vi "Set Annotation.vi"(8 "error in":errorcluster, 9 "XY Position":T1 caption="Position", 10 "Active Plot":u32, 11 "XY Plot":refnum<vi>) -> (0 "error out":errorcluster, 3 "XY Plot out":refnum<vi>)   [LabVIEW 2025, in "XY Plotter.lvlib" / "XY Plotter.lvclass"]
uses:
  XY Plotter.lvclass
  <vilib>/Utility/miscctls.llb/LVPointDoubleTypeDef.ctl
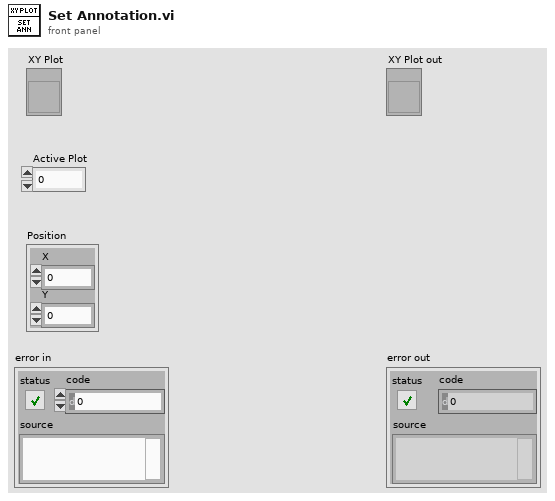
[diagram p1: front panel]
types:
  T1 = typedef "LVPointDoubleTypeDef.ctl" = cluster{"X":dbl, "Y":dbl}
  T2 = cluster{"Name":string, "Color":u32, "Style":u8, "Point Style":u8, "Name Visible":bool, "Allow Drag":bool, "Annotation Mode":u32, "Plot":i32, "Index":i32, "Position":cluster{"X":dbl, "Y":dbl}, "X Scale":u32, "Y Scale":u32, "Show Arrow":bool, "Lock Name":bool, "Plot Area":i32, "Label Offset":cluster{"X":dbl, "Y":dbl}}
  T3 = typedef "LVAnnotationListTypeDef.ctl" = cluster{"Name":string, "Color":u32, "Style":u8, "Point Style":u8, "Name Visible":bool, "Allow Drag":bool, "Annotation Mode":u32, "Plot":i32, "Index":i32, "Position":cluster{"X":dbl, "Y":dbl}, "X Scale":u32, "Y Scale":u32, "Show Arrow":bool, "Lock Name":bool, "Plot Area":i32, "Label Offset":cluster{"X":dbl, "Y":dbl}}[]
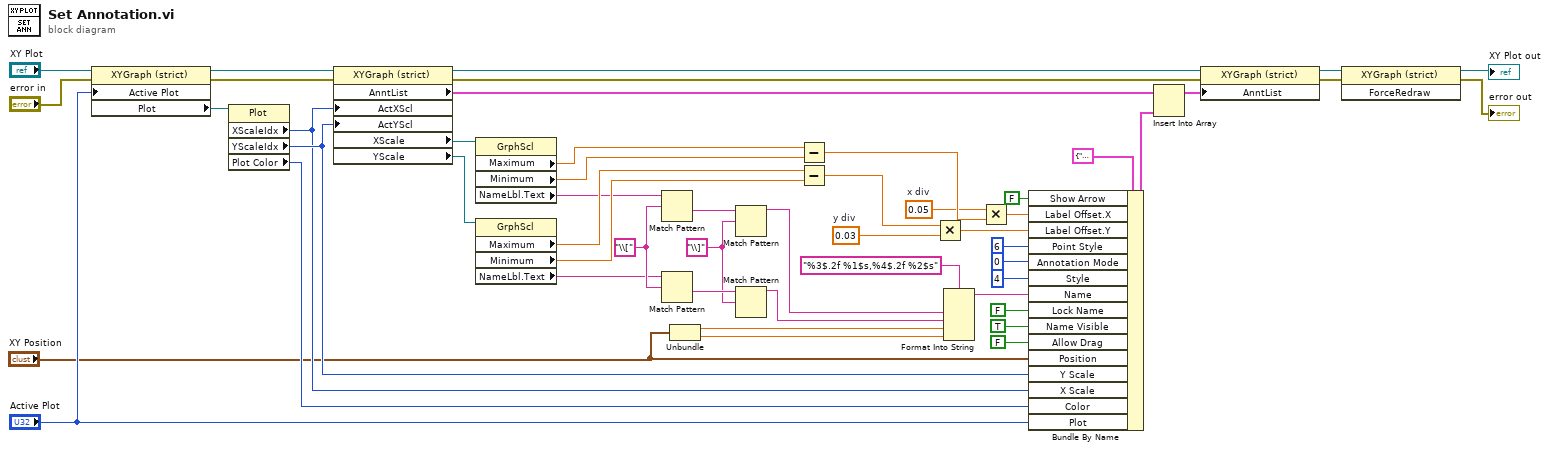
[diagram p0: block diagram]
diagram:
  w11 = "\\]" ("regular expression")
  w8 = "\\[" ("regular expression")
  w9 = 0.03  # y div
  w13 = 0.05  # x div
  n1 = property class="XYGraph (strict)"(reference="XY Plot", error in="error in", "Active Plot"="Active Plot") -> (reference out=w45:refnum<vi>, error out=w43:errorcluster, "Plot"=w35:refnum<vi>)
  n2 = property class="Plot"(reference=w35) -> ("XScaleIdx"=w32:u32, "YScaleIdx"=w33:u32, "Plot Color"=w34:u32)  [unwired: 1 in, 2 out]
  n3 = property class="XYGraph (strict)"(reference=w45, error in=w43, "ActXScl"=w32, "ActYScl"=w33) -> (reference out=w44:refnum<vi>, error out=w42:errorcluster, "AnntList"=w46:T3, "XScale"=w31:refnum<vi>, "YScale"=w30:refnum<vi>)
  n4 = property class="GrphScl"(reference=w31) -> ("Maximum"=w20:dbl, "Minimum"=w21:dbl, "NameLbl.Text"=w7:string)  [unwired: 1 in, 2 out]
  n5 = property class="GrphScl"(reference=w30) -> ("Maximum"=w22:dbl, "Minimum"=w23:dbl, "NameLbl.Text"=w6:string)  [unwired: 1 in, 2 out]
  n6 = Match Pattern(string=w7, regular expression=w8) -> (after substring=w17:string)  [unwired: 1 in, 3 out]
  n7 = Match Pattern(string=w6, regular expression=w8) -> (after substring=w16:string)  [unwired: 1 in, 3 out]
  n8 = Unbundle("XY Position") -> ("X"=w18:dbl, "Y"=w19:dbl)
  n9 = Match Pattern(string=w17, regular expression=w11) -> (before substring=w14:string)  [unwired: 1 in, 3 out]
  n10 = Match Pattern(string=w16, regular expression=w11) -> (before substring=w15:string)  [unwired: 1 in, 3 out]
  n11 = Subtract(x=w20, y=w21) -> (x-y=w24:dbl)
  n12 = Subtract(x=w22, y=w23) -> (x-y=w10:dbl)
  n13 = Multiply(x=w10, y=w9) -> (x*y=w29:dbl)
  n14 = Format Into String(format string="%3$.2f %1$s,%4$.2f %2$s", w14, w15, w18, w19) -> (resulting string=w25:string)  [unwired: 2 in, 1 out]
  n15 = Multiply(x=w13, y=w24) -> (x*y=w28:dbl)
  n16 = Bundle By Name(cluster=T2 {"Name"="", "Color"=0, "Style"=0, "Point Style"=0, "Name Visible"=FALSE, "Allow Drag"=FALSE, "Annotation Mode"=0, "Plot"=0, "Index"=0, "Position"={"X"=0.0, "Y"=0.0}, "X Scale"=0, "Y Scale"=0, "Show Arrow"=FALSE, "Lock Name"=FALSE, "Plot Area"=0, "Label Offset"={"X"=0.0, "Y"=0.0}} ("new element/subarray"), "Show Arrow"=FALSE, "Label Offset.X"=w28, "Label Offset.Y"=w29, "Point Style"=u8 6, "Annotation Mode"=u32 0, "Style"=u8 4, "Name"=w25, "Lock Name"=FALSE, "Name Visible"=TRUE, "Allow Drag"=FALSE, "Position"="XY Position", "Y Scale"=w33, "X Scale"=w32, "Color"=w34, "Plot"="Active Plot") -> (w47:T2)
  n17 = Insert Into Array(array=w46, new element=w47) -> (w51:T3)  [unwired: 1 in]
  n18 = property class="XYGraph (strict)"(reference=w44, error in=w42, "AnntList"=w51) -> (reference out=w4:refnum<vi>, error out=w3:errorcluster)
  n19 = invoke class="XYGraph (strict)" method="ForceRedraw"(reference=w4, error in=w3) -> (reference out=→"XY Plot out":refnum<vi>, error out=→"error out":errorcluster)  [unwired: 1 in, 1 out]
